vi "skeleton.vi"(11 "Inputs":string[](array[string])) -> (2 "Output/Failure":string, 3 "CLI Process Return Code":i32)   [LabVIEW 2026]
doc: "Slice 1.2 bridge skeleton. Connects to 127.0.0.1 on the port named in the rendezvous file (Inputs[0], default /tmp/lvmcp-skeleton-port.txt), then loops: read one length-prefixed frame (4-byte big-endian length, then the payload), answer one frame. The payload probe runs the VI Server constructs the bridge needs (Open Application Reference, Open VI Reference in that instance, Property Node, Invoke Node, Ctrl Val.Get and Ctrl Val.Set through Flatten To XML and Unflatten From XML) on the VI at Inputs[1] (default /tmp/fx/Target.vi). Any other payload is echoed. The loop ends on the first TCP error (66 is the peer closing, measured). Reentrant."
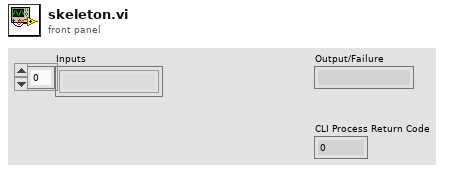
[diagram p1: front panel]
types:
  T1 = enum32{"Bad", "Idle", "Run top level", "Running"}
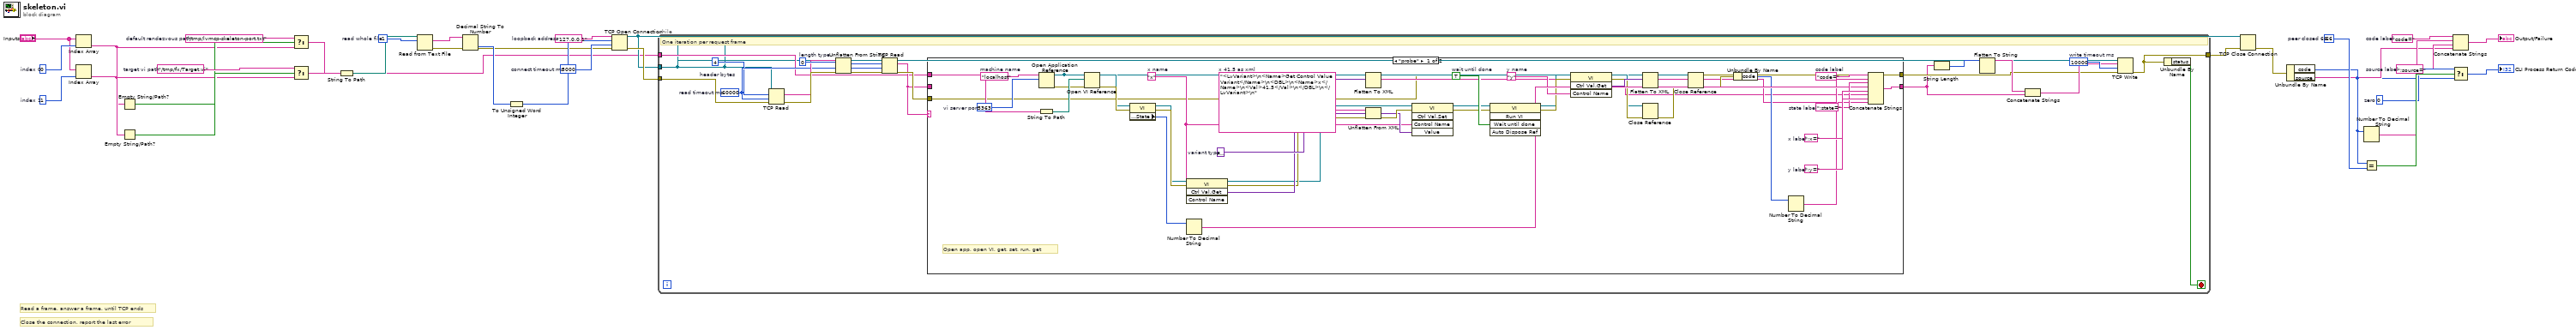
[diagram p0: block diagram]
diagram:
  w31 = 0  # zero
  w30 = 66  # peer closed 66
  w28 = ";source="  # source label
  w27 = "code="  # code label
  w17 = 5000  # connect timeout ms
  w16 = "127.0.0.1"  # loopback address
  w13 = -1  # read whole file
  w9 = "/tmp/fx/Target.vi"  # target vi path
  w4 = 1  # index 1
  w3 = 0  # index 0
  w2 = "/tmp/lvmcp-skeleton-port.txt"  # default rendezvous path
  # "Close the connection, report the last error"
  # "Read a frame, answer a frame, until TCP ends"
  n1 = Index Array(array="Inputs", index=w3) -> (element=w5:string)
  n2 = Index Array(array="Inputs", index=w4) -> (element=w6:string)
  n3 = Empty String/Path?(string/path=w5) -> (empty?=w7:bool)
  n4 = Empty String/Path?(string/path=w6) -> (empty?=w10:bool)
  n5 = Select(t=w2, s=w7, f=w5) -> (s? t:f=w8:string)
  n6 = Select(t=w9, s=w10, f=w6) -> (s? t:f=w11:string)
  n7 = String To Path(string=w8) -> (path=w12:path)
  n8 = Read from Text File(file (use dialog)=w12, count=w13) -> (text=w14:string, error out=w15:errorcluster)  [unwired: 2 in, 2 out]
  n9 = Decimal String To Number(string=w14) -> (number=w18:i32)  [unwired: 2 in, 1 out]
  n10 = To Unsigned Word Integer(number=w18) -> (unsigned 16bit integer=w19:u16)
  n11 = TCP Open Connection(address=w16, remote port or service name=w19, timeout ms (60000)=w17, error in (no error)=w15) -> (connection ID=w20:refnum<k5>, error out=w21:errorcluster)  [unwired: 1 in]
  n12 = while {
    tunnel: w11 -> [w36]
    tunnel: w20 -> [w34]
    tunnel: w21 -> [w35]
    tunnel: [w52] -> w22
    stop <- w53 stop-if-true
    w51 = 10000  # write timeout ms
    w41 = u32 0  # length type
    w38 = 60000  # read timeout ms
    w37 = 4  # header bytes
    # "One iteration per request frame"
    n13 = TCP Read(connection ID=w34, bytes to read=w37, error in (no error)=w35, 9:w38) -> (data out=w39:string, error out=w40:errorcluster)  [unwired: 1 in, 1 out]
    n14 = Unflatten From String(type=w41, binary string=w39, error in (no error)=w40) -> (value=w42:u32, error out=w43:errorcluster)  [unwired: 2 in, 1 out]
    n15 = TCP Read(connection ID=w34, bytes to read=w42, error in (no error)=w43, 9:w38) -> (data out=w44:string, error out=w45:errorcluster)  [unwired: 1 in, 1 out]
    n16 = case shown="\"b\", Default" w44 {
      tunnel: w36 -> [w55 _]
      tunnel: w44 -> [_ w95]
      tunnel: w45 -> [w54 w96]
      tunnel: [w54 w96] -> w47
      tunnel: [w94 w95] -> w46
      frame "probe" {
        w93 = ";y="  # y label
        w92 = ";x="  # x label
        w91 = ";state="  # state label
        w90 = "code="  # code label
        w80 = "y"  # y name
        w77 = TRUE  # wait until done
        w72 = variant  # variant type
        w71 = "<LvVariant>\n<Name>Get Control Value Variant</Name>\n<DBL>\n<Name>x</Name>\n<Val>41.5</Val>\n</DBL>\n</LvVariant>\n"  # x 41.5 as xml
        w66 = "x"  # x name
        w57 = u16 3363  # vi server port
        w56 = "localhost"  # machine name
        # "Open app, open VI, get, set, run, get"
        n17 = Open Application Reference(10:w57, 11:w56) -> (0:w59:errorcluster, 3:w58:refnum<vi>)  [unwired: 2 in]
        n18 = String To Path(string=w55) -> (path=w60:path)
        n19 = Open VI Reference(application reference (local)=w58, vi path=w60, error in (no error)=w59) -> (vi reference=w61:refnum<vi>, error out=w62:errorcluster)  [unwired: 3 in]
        n20 = property class="VI"(reference=w61, error in=w62) -> (reference out=w64:refnum<vi>, error out=w65:errorcluster, "Execution:State"=w63:T1)
        n21 = invoke class="VI" method="Ctrl Val.Get"(reference=w64, error in=w65, "Control Name"=w66) -> (reference out=w67:refnum<vi>, error out=w68:errorcluster, "Get Control Value Variant"=w69:variant)  [unwired: 1 in, 1 out]
        n22 = Number To Decimal String(number=w63) -> (decimal integer string=w89:string)  [unwired: 1 in]
        n23 = Flatten To XML(6:w69) -> (2:w70:string)
        n24 = Unflatten From XML(xml string=w71, type=w72, error in (no error)=w68) -> (value=w73:variant, error out=w74:errorcluster)
        n25 = invoke class="VI" method="Ctrl Val.Set"(reference=w67, error in=w74, "Control Name"=w66, "Value"=w73) -> (reference out=w75:refnum<vi>, error out=w76:errorcluster)  [unwired: 1 in, 3 out]
        n26 = invoke class="VI" method="Run VI"(reference=w75, error in=w76, "Wait until done"=w77) -> (reference out=w78:refnum<vi>, error out=w79:errorcluster)  [unwired: 2 in, 3 out]
        n27 = invoke class="VI" method="Ctrl Val.Get"(reference=w78, error in=w79, "Control Name"=w80) -> (reference out=w81:refnum<vi>, error out=w82:errorcluster, "Get Control Value Variant"=w83:variant)  [unwired: 1 in, 1 out]
        n28 = Flatten To XML(6:w83) -> (2:w84:string)
        n29 = Close Reference(reference=w81, error in (no error)=w82) -> (error out=w85:errorcluster)
        n30 = Close Reference(reference=w58, error in (no error)=w85) -> (error out=w86:errorcluster)
        n31 = Unbundle By Name(w86) -> ("code"=w87:i32)
        n32 = Number To Decimal String(number=w87) -> (decimal integer string=w88:string)  [unwired: 1 in]
        n33 = Concatenate Strings(w90, w88, w91, w89, w92, w70, w93, w84) -> (w94:string)
      }
      frame Default {
        # "Echo the payload unchanged"
      }
    }
    n34 = String Length(string=w46) -> (length=w48:i32)
    n35 = Flatten To String(anything=w48) -> (data string=w49:string)  [unwired: 3 in, 2 out]
    n36 = Concatenate Strings(w49, w46) -> (w50:string)
    n37 = TCP Write(connection ID=w34, data in=w50, error in (no error)=w47, 9:w51) -> (error out=w52:errorcluster)  [unwired: 2 out]
    n38 = Unbundle By Name(w52) -> ("status"=w53:bool)
  }
  n39 = TCP Close Connection(connection ID=w20, error in (no error)=w22) -> (error out=w23:errorcluster)  [unwired: 1 in, 1 out]
  n40 = Unbundle By Name(w23) -> ("code"=w24:i32, "source"=w25:string)
  n41 = Number To Decimal String(number=w24) -> (decimal integer string=w26:string)  [unwired: 1 in]
  n42 = Equal?(x=w24, y=w30) -> (x = y?=w32:bool[])
  n43 = Concatenate Strings(w27, w26, w28, w25) -> (→"Output/Failure":string)
  n44 = Select(t=w31, s=w32, f=w24) -> (s? t:f=→"CLI Process Return Code":i32)
